vi "start SA Measurement with OPC for single sweep.vi"(8 "error in (no error)":errorcluster, 9 "with OPC?":bool, 11 "FSV-40N in":refnum<class "FSV-40N.lvclass">) -> (0 "error out":errorcluster, 3 "FSV-40N out":refnum<class "FSV-40N.lvclass">)   [LabVIEW 2023, in "Spectrum Analyzer.lvlib" / "FSV-40N.lvclass"]
uses:
  FSV-40N.lvclass
  FSV-40N.lvclass/FSV-40N.ctl
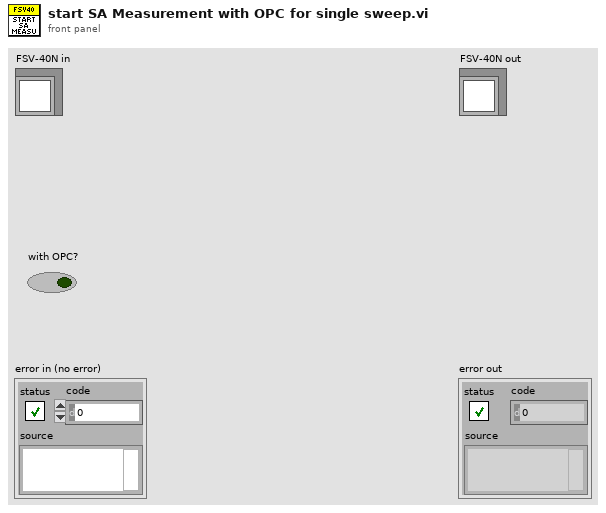
[diagram p1: front panel]
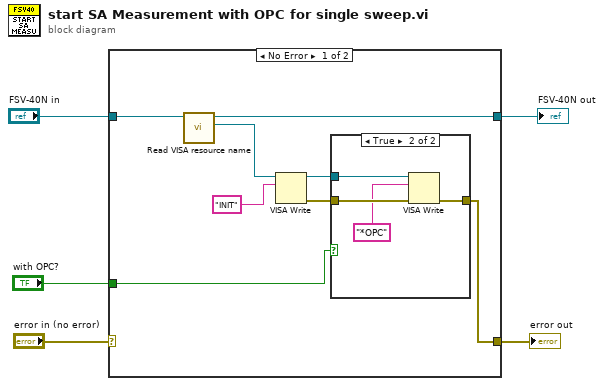
[diagram p0: block diagram]
diagram:
  n1 = case shown="No Error" "error in (no error)" {
    selector: "error in (no error)" -> [_ w19]
    tunnel: "FSV-40N in" -> [w13 w20]
    tunnel: [w7 w20] -> w3
    tunnel: [w6 w19] -> w2
    tunnel: "with OPC?" -> [w10 _]
    frame No Error {
      n2 = call "Read VISA resource name.vi"("FSV-40N in"=w13) -> ("VISA resource name"=w12:refnum<visa-resource-name>, "FSV-40N out"=w7:refnum<class "FSV-40N.lvclass">)  [unwired: 8 in, 1 out]
      n3 = VISA Write(VISA resource name=w12, write buffer="INIT") -> (VISA resource name out=w9:refnum<visa-resource-name>, error out=w8:errorcluster)  [unwired: 1 in, 1 out]
      n4 = case shown="True" w10 {
        tunnel: w9 -> [_ w18]
        tunnel: w8 -> [w14 w17]
        tunnel: [w14 w15] -> w6
        frame False {
        }
        frame True {
          n5 = VISA Write(VISA resource name=w18, write buffer="*OPC", error in (no error)=w17) -> (error out=w15:errorcluster)  [unwired: 2 out]
        }
      }
    }
    frame Error {
    }
  }
  "error out" <- w2
  "FSV-40N out" <- w3
